vi "check-broken.vi"(11 "error in":errorcluster) -> (15 "error out":errorcluster)   [LabVIEW 2020]
doc: "lvpm helper. Opens every VI listed in Files to check (one absolute path per line, CRLF or LF, empty lines ignored), reads its Execution State and closes it again - never saves, runs or shows a checked VI. Broken returns, one per line (LF), every path that is not executable or failed to open. Done turns true as the very last step."
panel:
  out "Done":bool
  out "Broken":string
  in  "Files to check":string
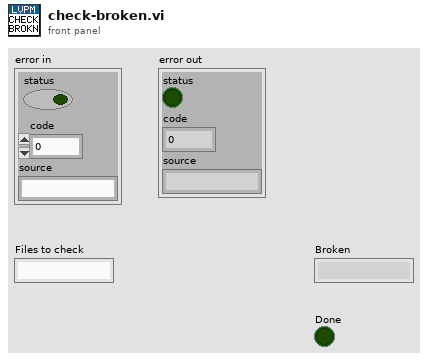
[diagram p1: front panel]
types:
  T1 = enum32{"Bad", "Idle", "Run top level", "Running"}
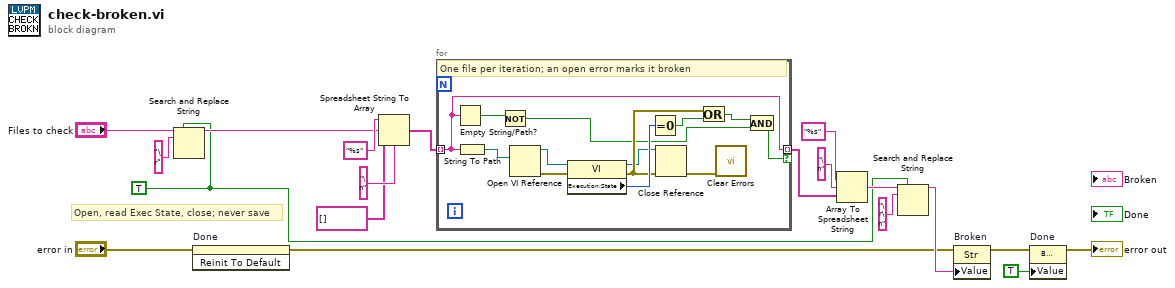
[diagram p0: block diagram]
diagram:
  w6 = TRUE ("replace all?")
  # "Open, read Exec State, close; never save"
  n1 = Search and Replace String(replace all?=w6, input string="Files to check", search string="\r") -> (result string=w7:string)  [unwired: 5 in, 3 out]
  n2 = invoke on="Done" class="Bool (strict)" method="Reinit To Default"(error in="error in") -> (error out=w4:errorcluster)  [unwired: 2 in, 2 out]
  n3 = Spreadsheet String To Array(delimiter (Tab)="\n", format string="%s", spreadsheet string=w7, array type (2D Dbl)=string[] []) -> (array=w11:string[])
  n4 = for {
    tunnel: w11 -> [w20] mode=indexing
    tunnel: [w20] -> w12 mode=indexing if=w31
    # "One file per iteration; an open error marks it broken"
    n5 = Empty String/Path?(string/path=w20) -> (empty?=w21:bool)
    n6 = String To Path(string=w20) -> (path=w23:path)
    n7 = Not(x=w21) -> (.not. x?=w22:bool)
    n8 = Open VI Reference(vi path=w23) -> (vi reference=w24:refnum<vi>, error out=w25:errorcluster)  [unwired: 5 in]
    n9 = property class="VI"(reference=w24, error in=w25) -> (reference out=w26:refnum<vi>, error out=w27:errorcluster, "Execution:State"=w28:T1)
    n10 = Equal To 0?(x=w28) -> (x = 0?=w29:bool)
    n11 = Close Reference(reference=w26, error in (no error)=w27) -> (error out=w32:errorcluster)
    n12 = Or(x=w27, y=w29) -> (x .or. y?=w30:bool)
    n13 = call <vilib>:"Clear Errors.vi"("error in (no error)"=w32) -> ()  [unwired: 5 in, 2 out]
    n14 = And(x=w30, y=w22) -> (x .and. y?=w31:bool)
  }
  n15 = Array To Spreadsheet String(delimiter (Tab)="\n", array=w12, 3:"%s" ("format string")) -> (spreadsheet string=w15:string)
  n16 = Search and Replace String(replace all?=w6, input string=w15, search string="\r\n") -> (result string=w17:string)  [unwired: 5 in, 3 out]
  n17 = property on="Broken" class="Str"(error in=w4, "Value"=w17) -> (error out=w18:errorcluster)  [unwired: 1 in, 1 out]
  n18 = property on="Done" class="Bool (strict)"(error in=w18, "Value"=TRUE) -> (error out=→"error out":errorcluster)  [unwired: 1 in, 1 out]
